vi "TARGET_856.vi"() -> ()   [LabVIEW 2018]
uses:
  <vilib>/Platform/TimedLoop/XDataNode/timing_clust.ctl
  <vilib>/Platform/TimedLoop/XDataNode/nitl_modes.ctl
  <vilib>/Platform/TimedLoop/XDataNode/wakeup.ctl
  <vilib>/rvi/eio/common/nirviEmuTemplateMethod_errors.vi
  <vilib>/rvi/Emulation/niFpgaGetClockAttributes.vi
  <vilib>/rvi/Emulation/niFpgaSctlEmulationGetInTimedLoop.vi
  <vilib>/rvi/Emulation/niFpgaEmulationReportErrorSimple.vi
  <vilib>/rvi/Emulation/niFpgaProcessEmulError.vi
  <vilib>/rvi/Emulation/niFpgaCriticalErrorInLSC.vi
  <vilib>/rvi/interface/RandomDataEmulation/niFpgaRandomDataHandleErrors.vi
  <vilib>/eio/EIONode/EIONode.xnode
  <vilib>/Platform/TimedLoop/XDataNode/XDataNode.xnode
  <vilib>/rvi/DataTransferAndStorage/Container/XNode/niFpgaContainer.xnode
  <vilib>/rvi/interface/RandomDataEmulation/nirviRandomDataFpgaReadWriteTemplate.vi
  <vilib>/Platform/TimedLoop/XDataNode/XDNodeRunTimeDep.lvlib
panel:
  in  "LED":bool
  in  "VINR":bool
  out "READ":bool[](array[boolean])
  in  "Write Data":bool[](array[boolean])=[FALSE, FALSE, FALSE, FALSE, FALSE, FALSE, FALSE, FALSE, FALSE]
  in  "Enum":T1(ring)=enum."GREEN OFF"
  in  "Read(T)/Write(F)":bool
  in  "Command array":bool[](array[boolean])=[FALSE, FALSE, FALSE, FALSE, FALSE, FALSE, FALSE, FALSE, FALSE, FALSE, FALSE, FALSE, FALSE, FALSE, FALSE, FALSE, FALSE]
  in  "Конфигурация":bool
  in  "Остановка основного цикла":bool
  in  "Линейки":bool
  in  "Между кадрами":u8=1 caption="Между кадрами, мс"
  out "Элем.":u32
  out "Данные":u8
  in  "CDS1_1":u8=2
  in  "CDS1_2":u8=4
  in  "CDS2_1":u8=5
  in  "CDS2_2":u8=7
  in  "ADC_1":u8=2
  in  "ADC_2":u8=7
  in  "RG_1":u8=1
  in  "RG_2":u8=2
  in  "PH21_1":u8=1
  in  "PH21_2":u8=6
  in  "PH11_1":u8=1
  in  "PH11_2":u8=6
  in  "HOR":u16=880
  in  "10":u8=10
  in  "LOW":u8=1
  in  "HIGH":u8=9
  in  "2017":u16=2017
  in  "PS1_2":u16=1809
  in  "PS1_1":u16=715
  in  "PS2_2":u16=1151
  in  "PS2_1":u16=496
  in  "PS3_2":u16=1589
  in  "PS3_1":u16=934
  in  "PS4_2":u16=1371
  in  "PS4_1":u16=277
  in  "Сколько строк?":i32=110
  in  "Кадр в FIFO":bool
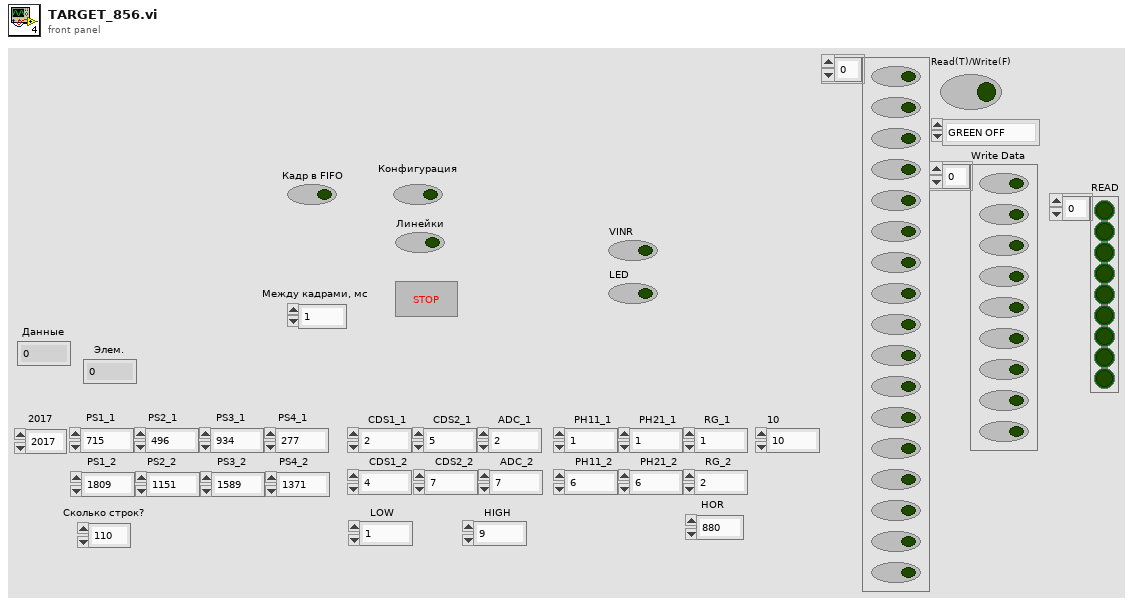
[diagram p1: front panel]
types:
  T1 = enum16{"Configuration", "MUX", "RED PGA", "GREEN PGA", "BLUE PGA", "RED OFF", "GREEN OFF", "BLUE OFF"}
  T2 = typedef "XDNodeRunTimeDep.lvlib/timing_clust.ctl" = cluster{"Expected End [f-1]":u64, "Actual End [f-1]":u64, "Finished Late? [f-1]":bool, "Expected End [i-1]":u64, "Actual End [i-1]":u64, "Finished Late? [i-1]":bool, "Expected Start [i]":u64, "Actual Start [i]":u64, "Expected Start [f]":u64, "Actual Start [f]":u64, "Source Name":string, "Structure Name":string, "Period":i64, "Deadline":i64, "Offset":i64, "Start":i64, "Priority":i32, "Timeout":i32, "Mode":T3, "Wakeup Reason":T4, "Error":errorcluster, "Source Type":string, "Secondary Source Type":string, "Global End Time":u64, "Global Start Time":u64, "Frame Duration":u64, "Iteration Duration":u64, "Assigned CPU":i32, "I/O Scan Engine Mode":u32}
  T3 = typedef "XDNodeRunTimeDep.lvlib/nitl_modes.ctl" = enum32{"No Change", "Process missed periods, maintain original phase", "Discard missed periods, maintain original phase", "Process missed periods, ignore original phase", "Discard missed periods, ignore original phase"}
  T4 = typedef "XDNodeRunTimeDep.lvlib/wakeup.ctl" = enum32{"Normal", "Aborted", "Asynchronous wakeup", "Timing source error", "Timed loop error", "Timeout"}
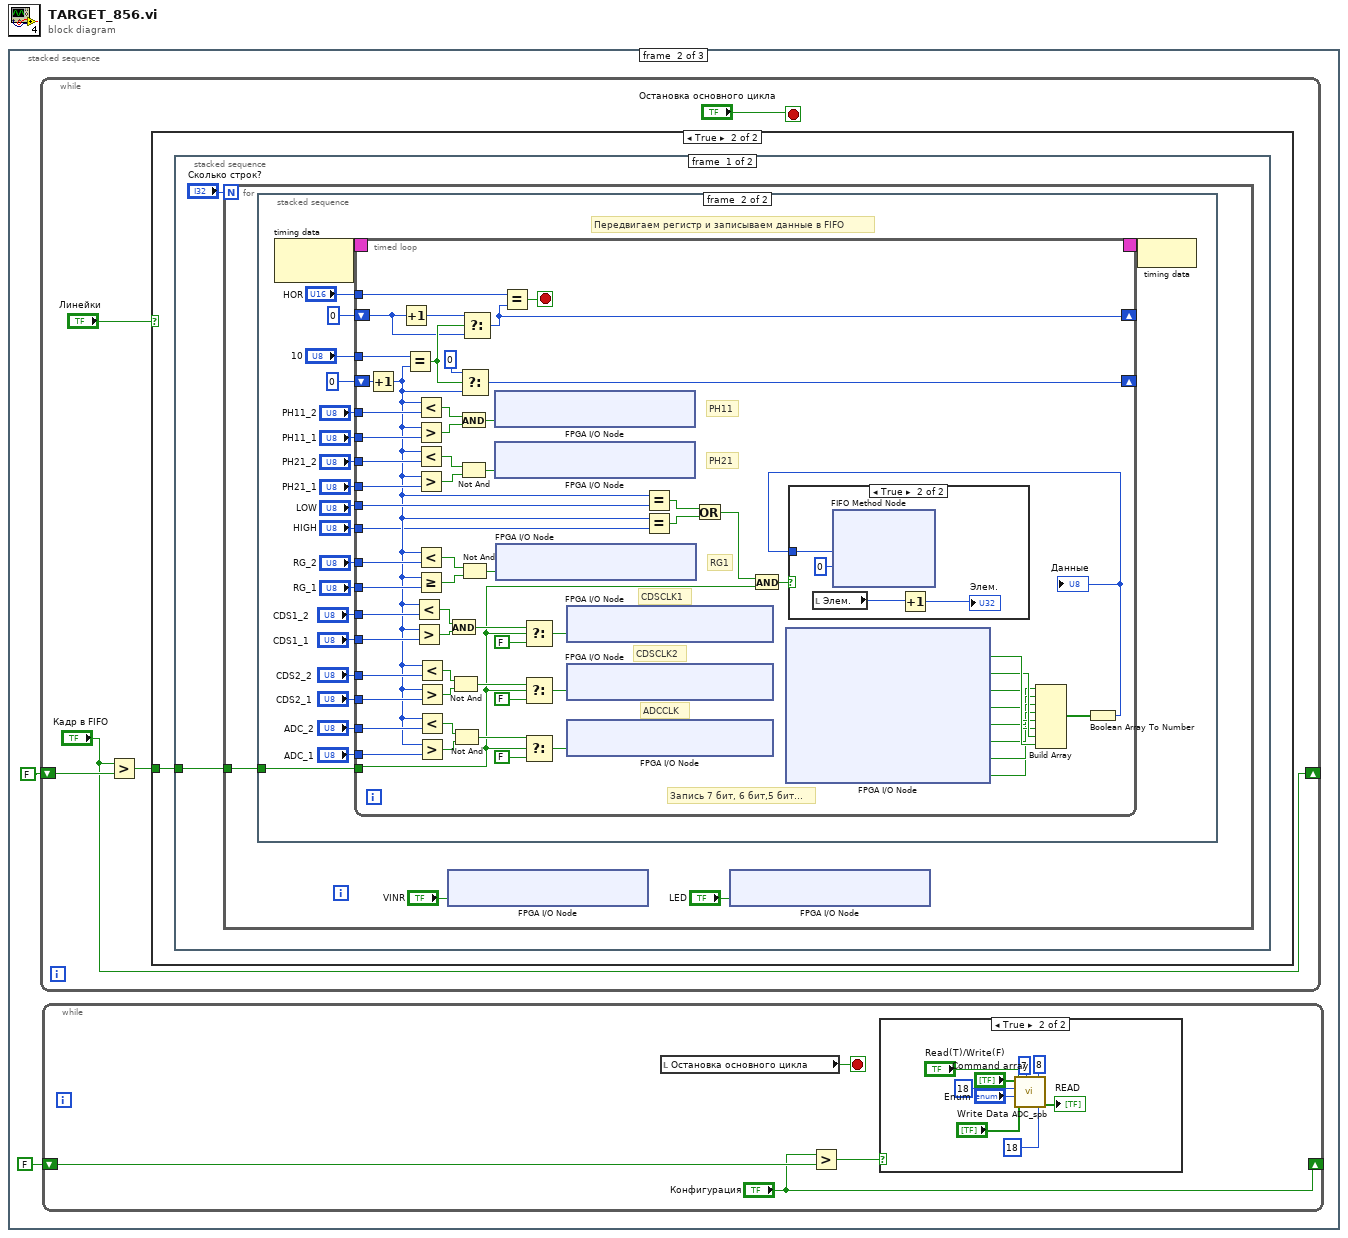
[diagram p0: block diagram]
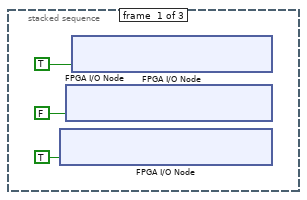
[diagram p2: hidden frame]
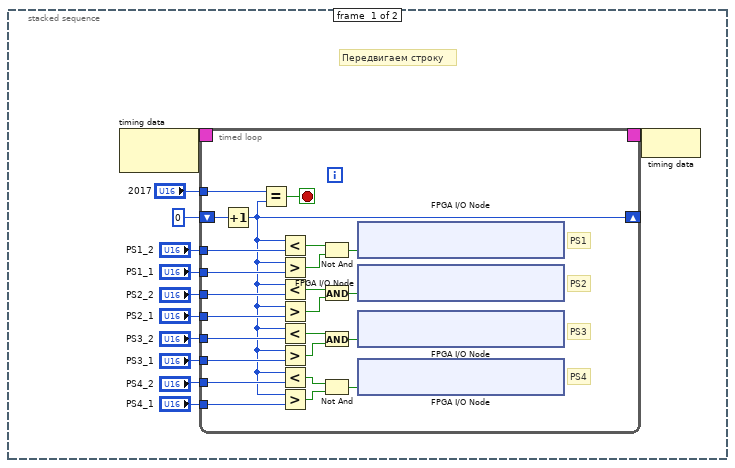
[diagram p4: hidden frame]
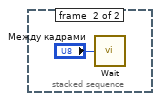
[diagram p6: hidden frame]
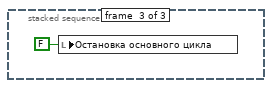
[diagram p8: hidden frame]
diagram:
  n1 = stacked-sequence {
    frame #0 {
      n2 = xnode "FPGA I/O Node"("IO Module\\DDCA_DIO16-23_WE"=TRUE) -> ()  [unwired: 1 in, 1 out]
      n3 = xnode "FPGA I/O Node"("IO Module\\DDCA_DIO8-15_WE"=FALSE) -> ()  [unwired: 1 in, 1 out]
      n4 = xnode "FPGA I/O Node"("IO Module\\DDCA_DIO0-7_WE"=TRUE) -> ()  [unwired: 1 in, 1 out]
    }
    frame #1 {
      n5 = while {
        shift-right: ["Кадр в FIFO"] -> _
        shift-left: FALSE ("Кадр в память") -> [w8]
        stop <- "Остановка основного цикла" stop-if-true
        n6 = Greater?(x="Кадр в FIFO", y=w8) -> (0:w6:bool)
        n7 = case shown="True" "Линейки" {
          tunnel: w6 -> [_ w11]
          frame False {
          }
          frame True {
            n8 = stacked-sequence {
              tunnel: w11 -> [w12 _]
              frame #0 {
                n9 = for {
                  N: "Сколько строк?" -> [_]
                  tunnel: w12 -> [w16]
                  n10 = stacked-sequence {
                    tunnel: w16 -> [_ w75]
                    frame #0 {
                      # "Передвигаем строку"
                      n11 = node-c288() -> (w28:T2)  [unwired: 1 in]
                      n12 = timed-loop {
                        timing: w28 -> [_]
                        timing-out: [_] -> w27
                        tunnel: "2017" -> [w51]
                        shift-right: [w29] -> _
                        shift-left: u16 0 -> [w52]
                        tunnel: "PS1_2" -> [w45]
                        tunnel: "PS1_1" -> [w44]
                        tunnel: "PS2_2" -> [w43]
                        tunnel: "PS2_1" -> [w42]
                        tunnel: "PS3_2" -> [w41]
                        tunnel: "PS3_1" -> [w40]
                        tunnel: "PS4_2" -> [w39]
                        tunnel: "PS4_1" -> [w38]
                        stop <- w50 stop-if-true
                        # "PS4"
                        # "PS3"
                        # "PS2"
                        # "PS1"
                        n13 = Increment(x=w52) -> (x+1=w29:u16)
                        n14 = Equal?(x=w51, y=w29) -> (x = y?=w50:bool)
                        n15 = Less?(x=w29, y=w45) -> (x < y?=w37:bool)
                        n16 = Greater?(x=w29, y=w44) -> (0:w36:bool)
                        n17 = Less?(x=w29, y=w43) -> (x < y?=w35:bool)
                        n18 = Greater?(x=w29, y=w42) -> (0:w34:bool)
                        n19 = Less?(x=w29, y=w41) -> (x < y?=w33:bool)
                        n20 = Greater?(x=w29, y=w40) -> (0:w32:bool)
                        n21 = Less?(x=w29, y=w39) -> (x < y?=w31:bool)
                        n22 = Greater?(x=w29, y=w38) -> (0:w30:bool)
                        n23 = Not And(1:w36, 2:w37) -> (0:w49:bool)
                        n24 = And(x=w35, y=w34) -> (x .and. y?=w48:bool)
                        n25 = And(x=w33, y=w32) -> (x .and. y?=w47:bool)
                        n26 = Not And(1:w30, 2:w31) -> (0:w46:bool)
                        n27 = xnode "FPGA I/O Node"("IO Module\\DDCA_DIO22_Write"=w49) -> ()  [unwired: 1 in, 1 out]
                        n28 = xnode "FPGA I/O Node"("IO Module\\DDCA_DIO21_Write"=w48) -> ()  [unwired: 1 in, 1 out]
                        n29 = xnode "FPGA I/O Node"("IO Module\\DDCA_DIO23_Write"=w47) -> ()  [unwired: 1 in, 1 out]
                        n30 = xnode "FPGA I/O Node"("IO Module\\DDCA_DIO20_Write"=w46) -> ()  [unwired: 1 in, 1 out]
                      }
                      n31 = node-c288(w27) -> ()
                    }
                    frame #1 {
                      # "Передвигаем регистр и записываем данные в FIFO"
                      n32 = node-c288() -> (w77:T2)  [unwired: 1 in]
                      n33 = timed-loop {
                        timing: w77 -> [_]
                        timing-out: [_] -> w76
                        tunnel: w75 -> [w116]
                        tunnel: "ADC_1" -> [w111]
                        tunnel: "ADC_2" -> [w110]
                        tunnel: "CDS2_1" -> [w109]
                        tunnel: "CDS2_2" -> [w108]
                        tunnel: "CDS1_1" -> [w107]
                        tunnel: "CDS1_2" -> [w106]
                        tunnel: "RG_1" -> [w105]
                        tunnel: "RG_2" -> [w104]
                        tunnel: "PH21_1" -> [w103]
                        tunnel: "PH21_2" -> [w102]
                        tunnel: "PH11_1" -> [w101]
                        tunnel: "PH11_2" -> [w100]
                        tunnel: "HOR" -> [w95]
                        shift-right: [w99] -> _
                        shift-left: u8 0 -> [w114]
                        tunnel: "10" -> [w112]
                        shift-right: [w94] -> _
                        shift-left: u16 0 ("Numeric") -> [w96]
                        tunnel: "LOW" -> [w89]
                        tunnel: "HIGH" -> [w87]
                        stop <- w93 stop-if-true
                        # "Запись 7 бит, 6 бит,5 бит..."
                        # "RG1"
                        # "PH21"
                        # "PH11"
                        # "ADCCLK"
                        # "CDSCLK2"
                        # "CDSCLK1"
                        n34 = Increment(x=w114) -> (x+1=w88:u8)
                        n35 = Increment(x=w96) -> (x+1=w97:u16)
                        n36 = Equal?(x=w112, y=w88) -> (x = y?=w98:bool)
                        n37 = Less?(x=w88, y=w106) -> (x < y?=w132:bool)
                        n38 = Greater?(x=w88, y=w107) -> (0:w131:bool)
                        n39 = Less?(x=w88, y=w100) -> (x < y?=w123:bool)
                        n40 = Greater?(x=w88, y=w101) -> (0:w122:bool)
                        n41 = Less?(x=w88, y=w102) -> (x < y?=w121:bool)
                        n42 = Greater?(x=w88, y=w103) -> (0:w120:bool)
                        n43 = Less?(x=w88, y=w104) -> (x < y?=w119:bool)
                        n44 = Greater Or Equal?(x=w88, y=w105) -> (x >= y?=w118:bool)
                        n45 = Less?(x=w88, y=w108) -> (x < y?=w129:bool)
                        n46 = Greater?(x=w88, y=w109) -> (0:w130:bool)
                        n47 = Less?(x=w88, y=w110) -> (x < y?=w128:bool)
                        n48 = Greater?(x=w88, y=w111) -> (0:w127:bool)
                        n49 = And(x=w132, y=w131) -> (x .and. y?=w135:bool)
                        n50 = Not And(1:w130, 2:w129) -> (0:w136:bool)
                        n51 = Not And(1:w127, 2:w128) -> (0:w137:bool)
                        n52 = And(x=w123, y=w122) -> (x .and. y?=w126:bool)
                        n53 = Not And(1:w120, 2:w121) -> (0:w125:bool)
                        n54 = Select(t=u8 0, s=w98, f=w88) -> (s? t:f=w99:u8)
                        n55 = Not And(1:w118, 2:w119) -> (0:w124:bool)
                        n56 = Select(t=w97, s=w98, f=w96) -> (s? t:f=w94:u16)
                        n57 = xnode "FPGA I/O Node"("IO Module\\DDCA_DIO4_Write"=w126) -> ()  [unwired: 1 in, 1 out]
                        n58 = xnode "FPGA I/O Node"("IO Module\\DDCA_DIO3_Write"=w125) -> ()  [unwired: 1 in, 1 out]
                        n59 = xnode "FPGA I/O Node"("IO Module\\DDCA_DIO2_Write"=w124) -> ()  [unwired: 1 in, 1 out]
                        n60 = Equal?(x=w95, y=w94) -> (x = y?=w93:bool)
                        n61 = Select(t=w135, s=w116, f=FALSE) -> (s? t:f=w133:bool)
                        n62 = Select(t=w136, s=w116, f=FALSE) -> (s? t:f=w134:bool)
                        n63 = Select(t=w137, s=w116, f=FALSE) -> (s? t:f=w141:bool)
                        n64 = xnode "FPGA I/O Node"("IO Module\\DDCA_DIO18_Write"=w133) -> ()  [unwired: 1 in, 1 out]
                        n65 = xnode "FPGA I/O Node"("IO Module\\DDCA_DIO17_Write"=w134) -> ()  [unwired: 1 in, 1 out]
                        n66 = xnode "FPGA I/O Node"("IO Module\\DDCA_DIO16_Write"=w141) -> ()  [unwired: 1 in, 1 out]
                        n67 = Equal?(x=w88, y=w89) -> (x = y?=w92:bool)
                        n68 = Equal?(x=w88, y=w87) -> (x = y?=w91:bool)
                        n69 = Or(x=w92, y=w91) -> (x .or. y?=w115:bool)
                        n70 = And(x=w115, y=w116) -> (x .and. y?=w117:bool)
                        n71 = xnode "FPGA I/O Node"() -> ("IO Module\\DDCA_DIO8_Read"=w86:bool, "IO Module\\DDCA_DIO9_Read"=w85:bool, "IO Module\\DDCA_DIO10_Read"=w84:bool, "IO Module\\DDCA_DIO11_Read"=w83:bool, "IO Module\\DDCA_DIO12_Read"=w82:bool, "IO Module\\DDCA_DIO13_Read"=w81:bool, "IO Module\\DDCA_DIO14_Read"=w80:bool, "IO Module\\DDCA_DIO15_Read"=w79:bool)  [unwired: 8 in, 8 out]
                        n72 = Build Array(w79, w80, w81, w82, w83, w84, w85, w86) -> (w78:bool[])
                        n73 = Boolean Array To Number(Boolean array=w78) -> (number=w90:u8)
                        "Данные" <- w90
                        n74 = case shown="True" w117 {
                          tunnel: w90 -> [_ w144]
                          frame False {
                          }
                          frame True {
                            n75 = local read "Элем."() -> (w143:u32)
                            n76 = xnode ("FIFO Method Node")("Element"=w144, "Timeout"=0) -> ()  [unwired: 1 in, 2 out]
                            n77 = Increment(x=w143) -> (x+1=→"Элем.":u32)
                          }
                        }
                      }
                      n78 = node-c288(w76) -> ()
                    }
                  }
                  n79 = xnode "FPGA I/O Node"("IO Module\\DDCA_DIO0_Write"="VINR") -> ()  [unwired: 1 in, 1 out]
                  n80 = xnode "FPGA I/O Node"("IO Module\\DDCA_DIO1_Write"="LED") -> ()  [unwired: 1 in, 1 out]
                }
              }
              frame #1 {
                n81 = call "Wait"("Count(mSec)"="Между кадрами") -> ()  [unwired: 1 out]
              }
            }
          }
        }
      }
      n82 = while {
        shift-right: ["Конфигурация"] -> _
        shift-left: FALSE ("Конфигурация") -> [w153]
        stop <- w154 stop-if-true
        n83 = local read "Остановка основного цикла"() -> (w154:bool)
        n84 = Greater?(x="Конфигурация", y=w153) -> (0:w151:bool)
        n85 = case shown="True" w151 {
          frame False {
          }
          frame True {
            n86 = call "ADC_spb.vi"(1:"18_1"=i8 18 ("18_1"), 2:"18_1"=i8 18 ("18_1"), "8"=i8 8, "7"=i8 7, "Write Data"="Write Data", "Enum"="Enum", "Read(T)/Write(F)"="Read(T)/Write(F)", "Command array"="Command array") -> ("READ"=→"READ":bool[])
          }
        }
      }
    }
    frame #2 {
      n87 = local write "Остановка основного цикла"(FALSE ("Остановка основного цикла")) -> ()
    }
  }
